vi "joystickAcquire.vi"(0 "device ID":refnum<k1>, 5 "error in (no error)":errorcluster) -> (15 "axis info":T1, 16 "button info":T3, 17 "direction info":T2, 19 "error out":errorcluster)   [LabVIEW 2026]
doc: "<p>Returns data about the device connected to the computer. Wire data to the <strong>device ID</strong> input to determine the polymorphic instance to use or <a href=\"nihelplauncher://docs/csh?context=lvcore_lvhowto_selectingdefaultinstpolyvi\">manually select</a> the instance.</p>"
uses:
  LabVIEW Data/libDS4LabVIEW.dylib
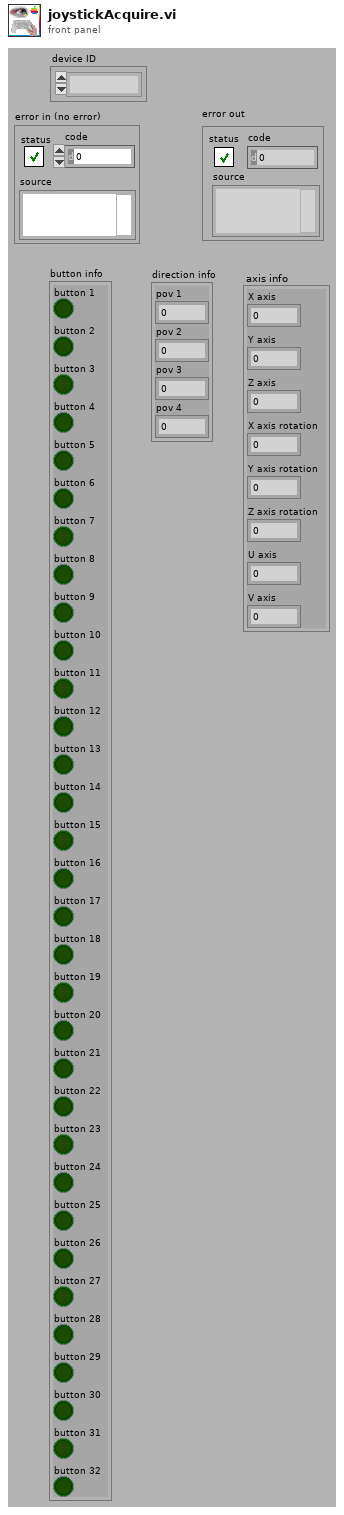
[diagram p1: front panel]
types:
  T1 = cluster{"X axis":i32, "Y axis":i32, "Z axis":i32, "X axis rotation":i32, "Y axis rotation":i32, "Z axis rotation":i32, "U axis":i32, "V axis":i32}
  T2 = cluster{"pov 1":i32, "pov 2":i32, "pov 3":i32, "pov 4":i32}
  T3 = cluster{"button 1":bool, "button 2":bool, "button 3":bool, "button 4":bool, "button 5":bool, "button 6":bool, "button 7":bool, "button 8":bool, "button 9":bool, "button 10":bool, "button 11":bool, "button 12":bool, "button 13":bool, "button 14":bool, "button 15":bool, "button 16":bool, "button 17":bool, "button 18":bool, "button 19":bool, "button 20":bool, "button 21":bool, "button 22":bool, "button 23":bool, "button 24":bool, "button 25":bool, "button 26":bool, "button 27":bool, "button 28":bool, "button 29":bool, "button 30":bool, "button 31":bool, "button 32":bool}
  T4 = cluster{bool, bool, bool, bool, bool, bool, bool, bool, bool, bool, bool, bool, bool, bool, bool, bool, bool, bool, bool, bool, bool, bool, bool, bool, bool, bool, bool, bool, bool, bool, bool, bool}
  T5 = cluster{"axis[0]":sgl, "axis[1]":sgl, "axis[2]":sgl, "axis[3]":sgl, "axis[4]":sgl, "axis[5]":sgl, "axis[6]":sgl, "axis[7]":sgl}
  T6 = cluster{"[0]":bool, "[1]":bool, "[2]":bool, "[3]":bool, "[4]":bool, "[5]":bool, "[6]":bool, "[7]":bool, "[8]":bool, "[9]":bool, "[10]":bool, "[11]":bool, "[12]":bool, "[13]":bool, "[14]":bool, "[15]":bool, "[16]":bool, "[17]":bool, "[18]":bool, "[19]":bool, "[20]":bool, "[21]":bool, "[22]":bool, "[23]":bool, "[24]":bool, "[25]":bool, "[26]":bool, "[27]":bool, "[28]":bool, "[29]":bool, "[30]":bool, "[31]":bool}
  T7 = cluster{"directions[0]":i32, "directions[1]":i32, "directions[2]":i32, "directions[3]":i32}
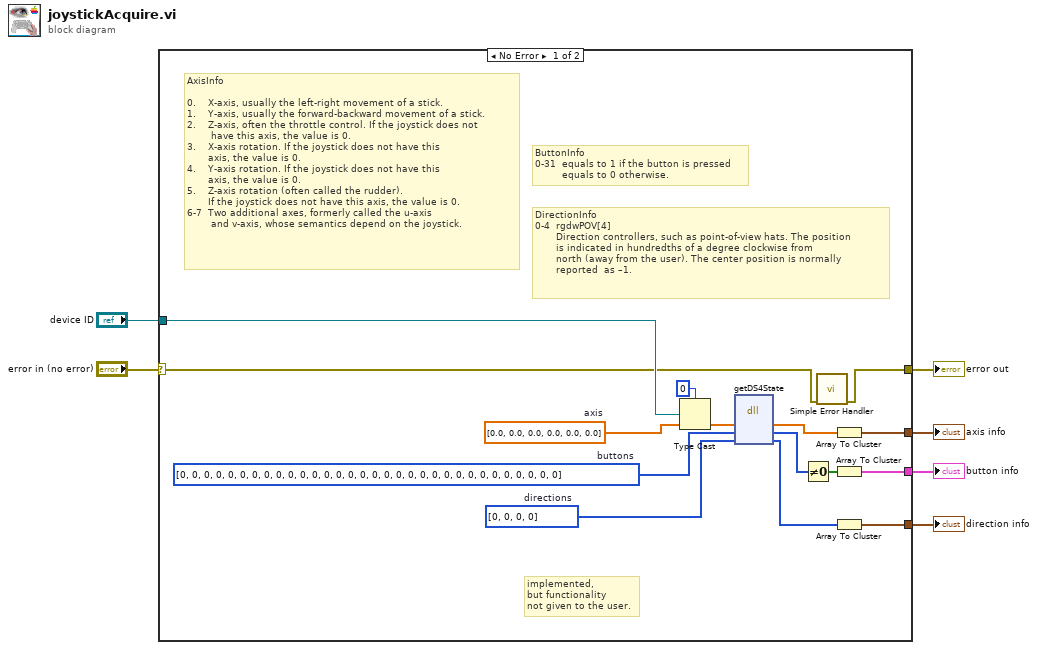
[diagram p0: block diagram]
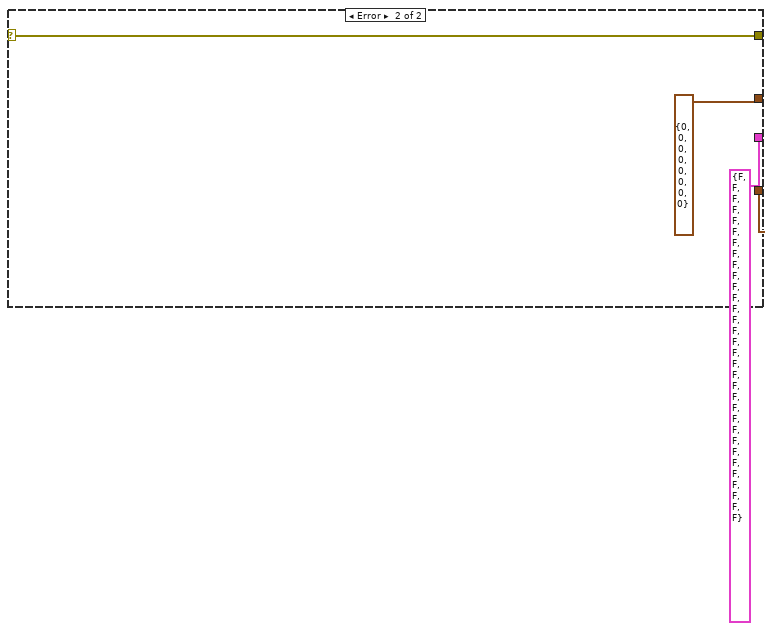
[diagram p2: hidden frame]
diagram:
  n1 = case shown="No Error" "error in (no error)" {
    selector: "error in (no error)" -> [w8 w21]
    tunnel: [w7 w21] -> w6
    tunnel: [w12 cluster{i32, i32, i32, i32} {0, 0, 0, 0}] -> w5
    tunnel: [w11 T4 {FALSE, FALSE, FALSE, FALSE, FALSE, FALSE, FALSE, FALSE, FALSE, FALSE, FALSE, FALSE, FALSE, FALSE, FALSE, FALSE, FALSE, FALSE, FALSE, FALSE, FALSE, FALSE, FALSE, FALSE, FALSE, FALSE, FALSE, FALSE, FALSE, FALSE, FALSE, FALSE}] -> w4
    tunnel: [w10 cluster{i32, i32, i32, i32, i32, i32, i32, i32} {0, 0, 0, 0, 0, 0, 0, 0}] -> w3
    tunnel: "device ID" -> [w9 _]
    frame No Error {
      w18 = i32[] [0, 0, 0, 0]  # directions
      w19 = i8[] [0, 0, 0, 0, 0, 0, 0, 0, 0, 0, 0, 0, 0, 0, 0, 0, 0, 0, 0, 0, 0, 0, 0, 0, 0, 0, 0, 0, 0, 0, 0, 0]  # buttons
      w20 = dbl[] [0.0, 0.0, 0.0, 0.0, 0.0, 0.0]  # axis
      # "implemented,\nbut functionality\nnot given to the user."
      # "DirectionInfo\n0-4  rgdwPOV[4] \n       Direction controllers, such as point-of-view hats. The position \n       is indicated in hundredths of a degree clockwise from\n       north (away from the user). The center position is normally \n       reported  as –1."
      # "ButtonInfo\n0-31  equals to 1 if the button is pressed\n         equals to 0 otherwise."
      # "AxisInfo \n\n0.    X-axis, usually the left-right movement of a stick. \n1.    Y-axis, usually the forward-backward movement of a stick. \n2.    Z-axis, often the throttle control. If the joystick does not \n        have this axis, the value is 0. \n3.    X-axis rotation. If the joystick does not have this \n       axis, the value is 0. \n4.    Y-axis rotation. If the joystick does not have this \n       axis, the value is 0. \n5.    Z-axis rotation (often called the rudder). \n       If the joystick does not have this axis, the value is 0. \n6-7  Two additional axes, formerly called the u-axis\n        and v-axis, whose semantics depend on the joystick."
      n2 = Type Cast(type=0, x=w9) -> ()  [unwired: 1 out]
      n3 = dll-call lib="Users/eira/Documents/LabVIEW Data/libDS4LabVIEW.dylib" fn="getDS4State"("axis"=w20, "buttons"=w19, "directions"=w18) -> ("axis"=w15:sgl[], "buttons"=w17:i32[], "directions"=w13:i32[])  [unwired: 4 in, 2 out]
      n4 = Not Equal To 0?(x=w17) -> (x != 0?=w14:bool[])
      n5 = call <vilib>:"Simple Error Handler.vi"("error in (no error)"=w8) -> ("error out"=w7:errorcluster)  [unwired: 4 in, 4 out]
      n6 = Array To Cluster(array=w15) -> (cluster=w10:T5)
      n7 = Array To Cluster(array=w14) -> (cluster=w11:T6)
      n8 = Array To Cluster(array=w13) -> (cluster=w12:T7)
    }
    frame Error {
    }
  }
  "error out" <- w6
  "direction info" <- w5
  "button info" <- w4
  "axis info" <- w3
